vi "set Marker Search Line.vi"(8 "error in (no error)":errorcluster, 10 "Marker Search Freq (Hz)":T1 {"Right Limit" format="%#_6p"; "Left Limit" format="%#_6p"}, 11 "FSV-40N in":refnum<class "FSV-40N.lvclass">) -> (0 "error out":errorcluster, 3 "FSV-40N out":refnum<class "FSV-40N.lvclass">)   [LabVIEW 2023, in "Spectrum Analyzer.lvlib" / "FSV-40N.lvclass"]
uses:
  FSV-40N.lvclass
  TYPE DEFINITION/TYPE Marker Search Limit Set.ctl
  FSV-40N.lvclass/FSV-40N.ctl
  Spectrum Analyzer.lvlib
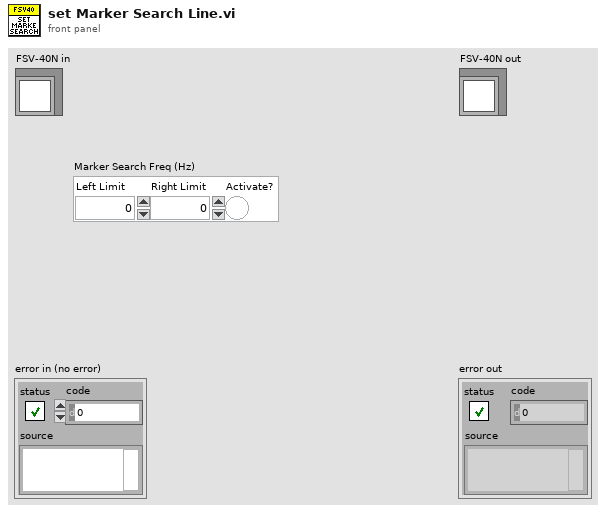
[diagram p1: front panel]
types:
  T1 = typedef "Spectrum Analyzer.lvlib/TYPE Marker Search Limit Set.ctl" = cluster{"Left Limit":dbl, "Right Limit":dbl, "Activate?":bool}
  T2 = typedef "Spectrum Analyzer.lvlib/TYPE Start and Stop Frequency.ctl" = cluster{"Start":dbl, "Stop":dbl}
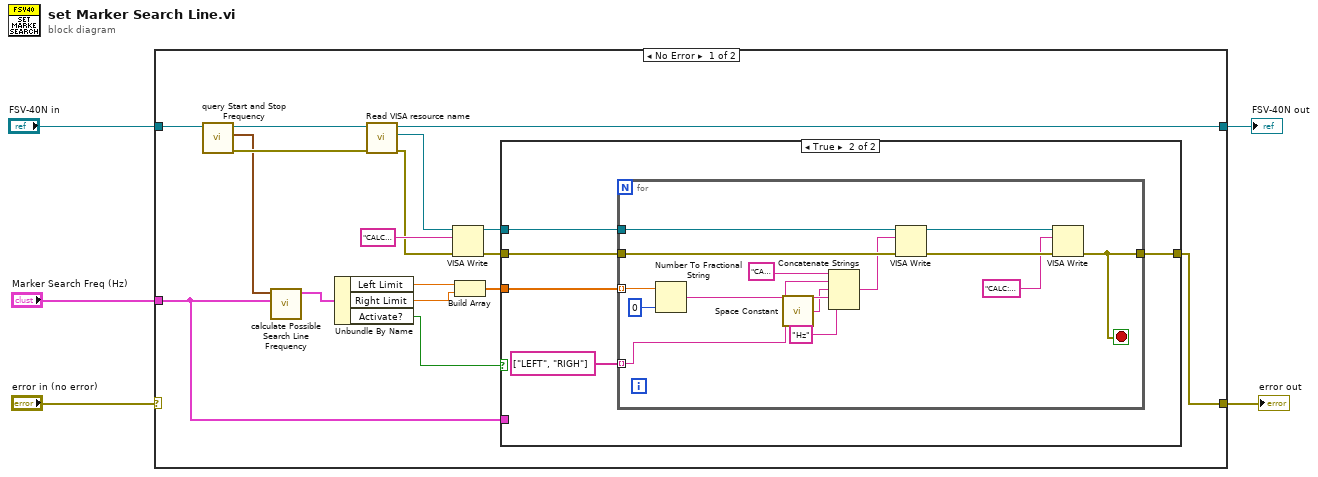
[diagram p0: block diagram]
diagram:
  n1 = case shown="No Error" "error in (no error)" {
    selector: "error in (no error)" -> [_ w43]
    tunnel: "FSV-40N in" -> [w15 w44]
    tunnel: [w22 w44] -> w3
    tunnel: [w20 w43] -> w2
    tunnel: "Marker Search Freq (Hz)" -> [w10 _]
    frame No Error {
      n2 = call-dynamic "query Start and Stop Frequency.vi"("FSV-40N in"=w15) -> ("error out"=w13:errorcluster, "Start/Stop Frequency(Hz)"=w11:T2, "FSV-40N out"=w14:refnum<class "FSV-40N.lvclass">)  [unwired: 8 in]
      n3 = call "calculate Possible Search Line Frequency.vi"("Marker Search Freq (Hz)"=w10, "Start/Stop Frequency(Hz)"=w11) -> ("Calculated Marker Search Freq (Hz)"=w9:T1)  [unwired: 9 in]
      n4 = Unbundle By Name(w9) -> ("Left Limit"=w8:dbl, "Right Limit"=w7:dbl, "Activate?"=w6:bool)
      n5 = call "Read VISA resource name.vi"("error in (no error)"=w13, "FSV-40N in"=w14) -> ("error out"=w12:errorcluster, "VISA resource name"=w18:refnum<visa-resource-name>, "FSV-40N out"=w22:refnum<class "FSV-40N.lvclass">)  [unwired: 7 in]
      n6 = VISA Write(VISA resource name=w18, write buffer="CALC:MARK:X:SLIM OFF", error in (no error)=w12) -> (VISA resource name out=w17:refnum<visa-resource-name>, error out=w16:errorcluster)  [unwired: 1 out]
      n7 = Build Array(w8, w7) -> (w21:dbl[])
      n8 = case shown="True" w6 {
        tunnel: w17 -> [_ w25]
        tunnel: w10 -> [_ _]
        tunnel: w21 -> [_ w28]
        tunnel: [w23 w26] -> w20
        tunnel: w16 -> [w23 w24]
        frame False {
        }
        frame True {
          n9 = for {
            tunnel: w28 -> [w40] mode=indexing
            tunnel: w25 -> [w42]
            tunnel: w24 -> [w41]
            tunnel: string[] ["LEFT", "RIGH"] -> [w38] mode=indexing
            tunnel: [w34] -> w26
            stop <- w34 stop-if-true
            n10 = Number To Fractional String(number=w40, precision (6)=i16 0) -> (F-format string=w37:string)  [unwired: 2 in]
            n11 = call <vilib>:"Space Constant.vi"() -> ("String"=w31:string)
            n12 = Concatenate Strings("CALC:MARK:X:SLIM:" ("string"), w38, w31, w37, "Hz" ("string")) -> (w29:string)
            n13 = VISA Write(VISA resource name=w42, write buffer=w29, error in (no error)=w41) -> (VISA resource name out=w36:refnum<visa-resource-name>, error out=w35:errorcluster)  [unwired: 1 out]
            n14 = VISA Write(VISA resource name=w36, write buffer="CALC:MARK:X:SLIM ON", error in (no error)=w35) -> (error out=w34:errorcluster)  [unwired: 2 out]
          }
        }
      }
    }
    frame Error {
    }
  }
  "error out" <- w2
  "FSV-40N out" <- w3
